vi "Recycle.vi"() -> ()   [LabVIEW 2026]
panel:
  out "Actions":T1
  out "Current Total ($)":dbl
  in  "Exit":bool
  in  "Receipt":bool
  in  "Sort":bool
  in  "Barcode":string(combo)
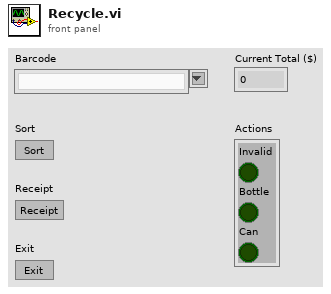
[diagram p1: front panel]
types:
  T1 = cluster{"Invalid":bool, "Bottle":bool, "Can":bool}
  T2 = cluster{"Reset":bool, "Delay Time (s)":dbl, "Total ($)":dbl, "Actions":cluster{"Invalid":bool, "Bottle":bool, "Can":bool}}
  T3 = enum16{"Initialize", "Read", "Sort", "Receipt", "Exit"}
  T4 = enum16{"open", "replace", "create", "open or create", "replace or create", "replace or create with confirmation"}
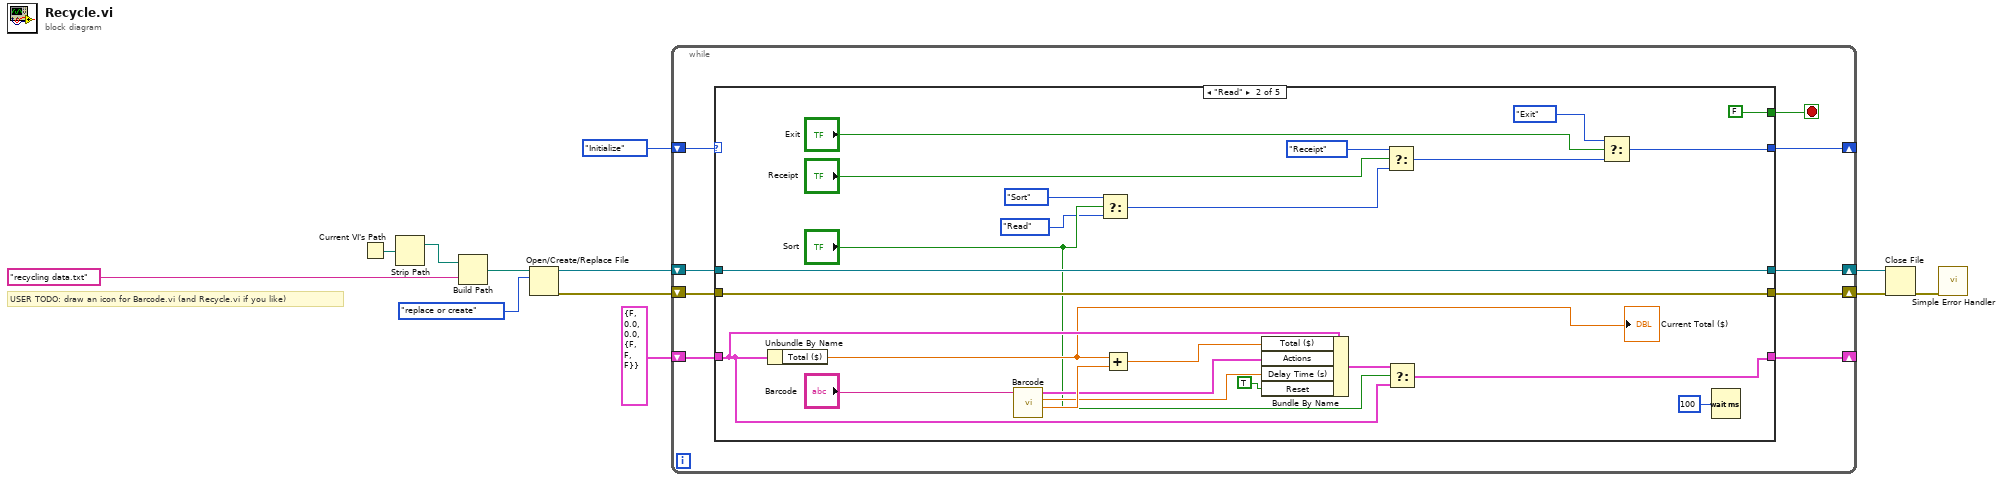
[diagram p0: block diagram]
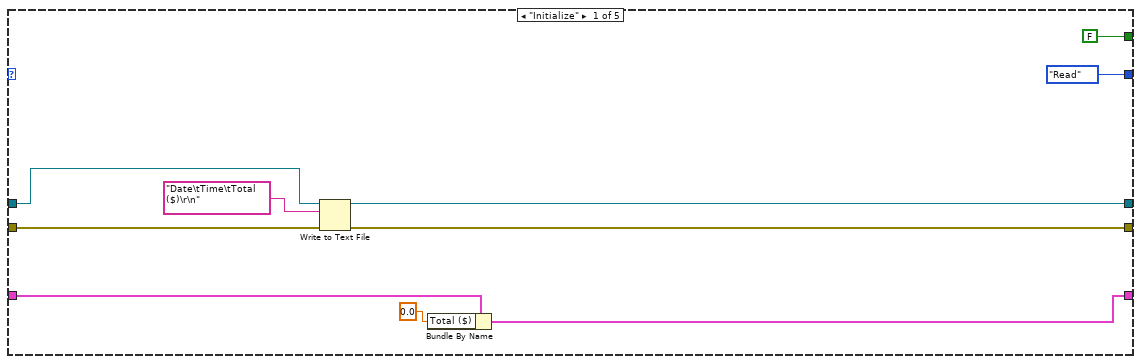
[diagram p2: hidden frame]
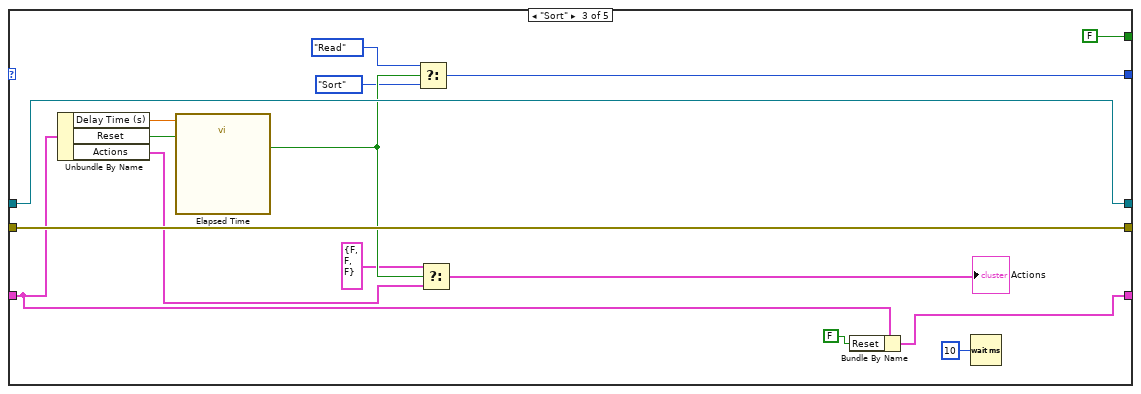
[diagram p3: hidden frame]
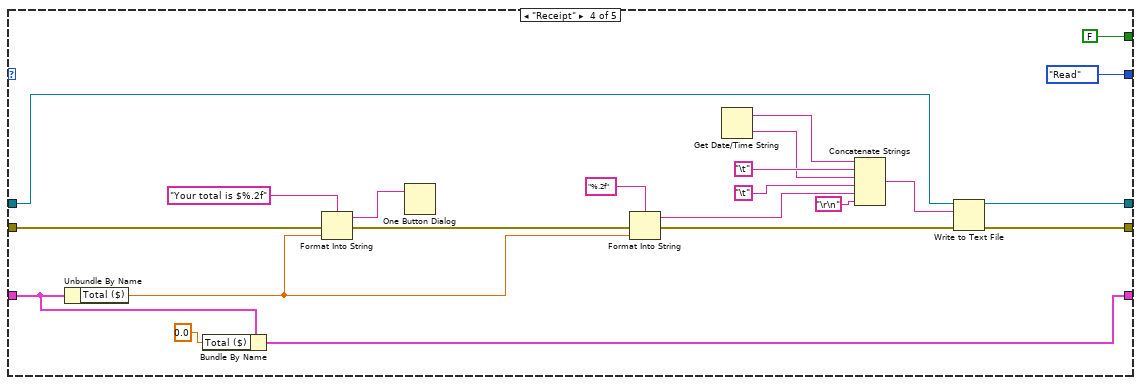
[diagram p4: hidden frame]
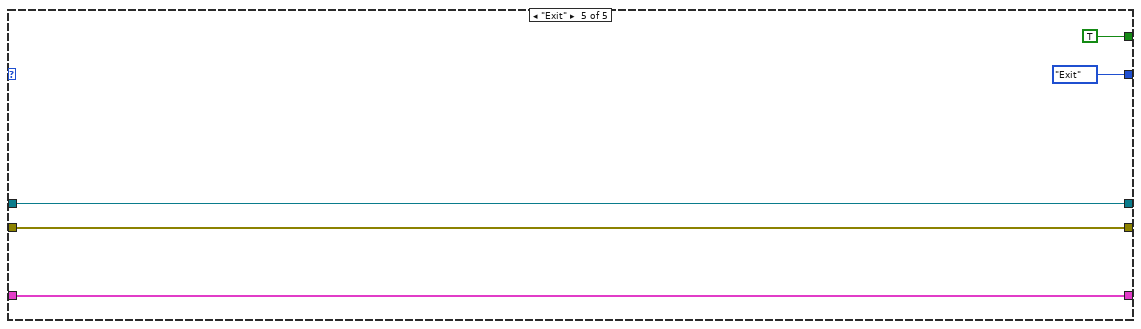
[diagram p5: hidden frame]
diagram:
  # "USER TODO: draw an icon for Barcode.vi (and Recycle.vi if you like)"
  n1 = Current VI's Path() -> (path=w12:path)
  n2 = Strip Path(path=w12) -> (stripped path=w11:path)  [unwired: 1 out]
  n3 = Build Path(base path=w11, name or relative path="recycling data.txt") -> (appended path=w9:path)
  n4 = Open/Create/Replace File(file path (use dialog)=w9, operation (0:open)=T4."replace or create") -> (refnum out=w5:refnum<file>, error out=w4:errorcluster)  [unwired: 4 in, 1 out]
  n5 = while {
    shift-right: [w14] -> _
    shift-left: T3."Initialize" ("State") -> [w21]
    shift-right: [w15] -> _
    shift-left: T2 {"Reset"=FALSE, "Delay Time (s)"=0.0, "Total ($)"=0.0, "Actions"={"Invalid"=FALSE, "Bottle"=FALSE, "Can"=FALSE}} ("Data") -> [w16]
    shift-right: [w18] -> w3
    shift-left: w5 -> [w20]
    shift-right: [w17] -> w2
    shift-left: w4 -> [w19]
    stop <- w13 stop-if-true
    n6 = case shown="\"Read\"" w21 {
      tunnel: w20 -> [w31 w55 w71 w80 w98]
      tunnel: w19 -> [w30 w54 w70 w90 w97]
      tunnel: [w28 w55 w71 w77 w98] -> w18
      tunnel: [w27 w54 w70 w76 w97] -> w17
      tunnel: w16 -> [w26 w52 w69 w93 w96]
      tunnel: [w24 w43 w65 w74 w96] -> w15
      tunnel: [T3."Read" ("State") w34 w58 T3."Read" ("State") T3."Exit" ("State")] -> w14
      tunnel: [FALSE FALSE FALSE FALSE TRUE] -> w13
      frame "Initialize" {
        n7 = Write to Text File(file (use dialog)=w31, text="Date\tTime\tTotal ($)\r\n", error in=w30) -> (refnum out=w28:refnum<file>, error out=w27:errorcluster)  [unwired: 1 in, 1 out]
        n8 = Bundle By Name(cluster=w26, "Total ($)"=0.0) -> (w24:T2)
      }
      frame "Read" {
        n9 = Unbundle By Name(w52) -> ("Total ($)"=w51:dbl)
        "Current Total ($)" <- w51
        n10 = call "Barcode.vi"("Barcode"="Barcode") -> ("Value ($)"=w50:dbl, "Delay Time (s)"=w47:dbl, "Actions"=w48:T1)  [unwired: 8 in]
        n11 = Select(t=T3."Sort" ("State"), s="Sort", f=T3."Read" ("State")) -> (s? t:f=w38:T3)
        n12 = Add(x=w51, y=w50) -> (x+y=w49:dbl)
        n13 = Bundle By Name(cluster=w52, "Total ($)"=w49, "Actions"=w48, "Delay Time (s)"=w47, "Reset"=TRUE) -> (w44:T2)
        n14 = Select(t=T3."Receipt" ("State"), s="Receipt", f=w38) -> (s? t:f=w35:T3)
        n15 = Select(t=w44, s="Sort", f=w52) -> (s? t:f=w43:T2)
        n16 = Select(t=T3."Exit" ("State"), s="Exit", f=w35) -> (s? t:f=w34:T3)
        n17 = Wait (ms)(milliseconds to wait=100) -> ()  [unwired: 1 out]
      }
      frame "Sort" {
        n18 = Unbundle By Name(w69) -> ("Delay Time (s)"=w68:dbl, "Reset"=w67:bool, "Actions"=w62:T1)
        n19 = call "Elapsed Time"("Time Target (s)"=w68, "Reset"=w67) -> ("Time has Elapsed"=w64:bool)  [unwired: 10 in, 7 out]
        n20 = Select(t=T3."Read" ("State"), s=w64, f=T3."Sort" ("State")) -> (s? t:f=w58:T3)
        n21 = Select(t=T1 {"Invalid"=FALSE, "Bottle"=FALSE, "Can"=FALSE} ("Actions 2"), s=w64, f=w62) -> (s? t:f=→"Actions":T1)
        n22 = Bundle By Name(cluster=w69, "Reset"=FALSE) -> (w65:T2)
        n23 = Wait (ms)(milliseconds to wait=10) -> ()  [unwired: 1 out]
      }
      frame "Receipt" {
        n24 = Unbundle By Name(w93) -> ("Total ($)"=w91:dbl)
        n25 = Bundle By Name(cluster=w93, "Total ($)"=0.0) -> (w74:T2)
        n26 = Format Into String(format string="Your total is $%.2f", error in=w90, w91) -> (resulting string=w89:string, error out=w87:errorcluster)  [unwired: 1 in]
        n27 = One Button Dialog(message=w89) -> ()  [unwired: 1 in, 1 out]
        n28 = Format Into String(format string="%.2f", error in=w87, w91) -> (resulting string=w82:string, error out=w78:errorcluster)  [unwired: 1 in]
        n29 = Get Date/Time String() -> (date string=w86:string, time string=w84:string)  [unwired: 3 in]
        n30 = Concatenate Strings(w86, "\t", w84, "\t", w82, "\r\n") -> (w79:string)
        n31 = Write to Text File(file (use dialog)=w80, text=w79, error in=w78) -> (refnum out=w77:refnum<file>, error out=w76:errorcluster)  [unwired: 1 in, 1 out]
      }
      frame "Exit" {
      }
    }
  }
  n32 = Close File(refnum=w3, error in=w2) -> (error out=w1:errorcluster)  [unwired: 1 out]
  n33 = call <vilib>:"Simple Error Handler.vi"("error in (no error)"=w1) -> ()  [unwired: 4 in, 5 out]
